vi "new-cacode.vi"() -> ()   [LabVIEW 2023]
uses:
  <vilib>/Utility/file.llb/Read Delimited Spreadsheet (string).vi
panel:
  out "all rows":string[][](array[string])
  in  "stop":bool
  in  "Run PRN Generator":bool
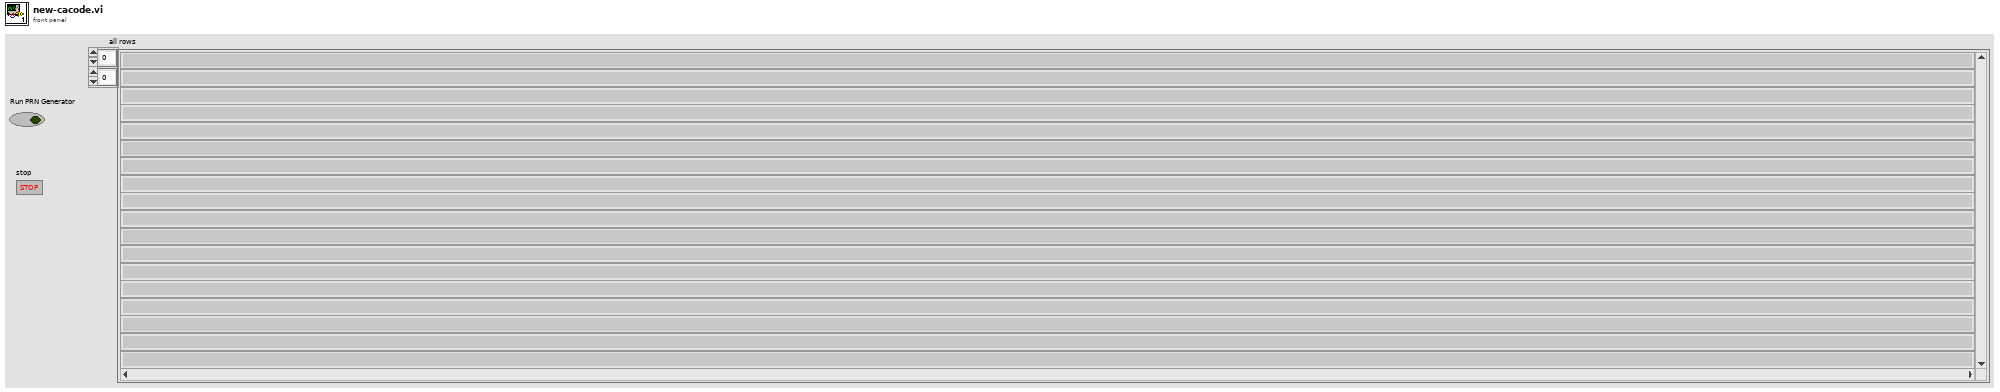
[diagram p1: front panel]
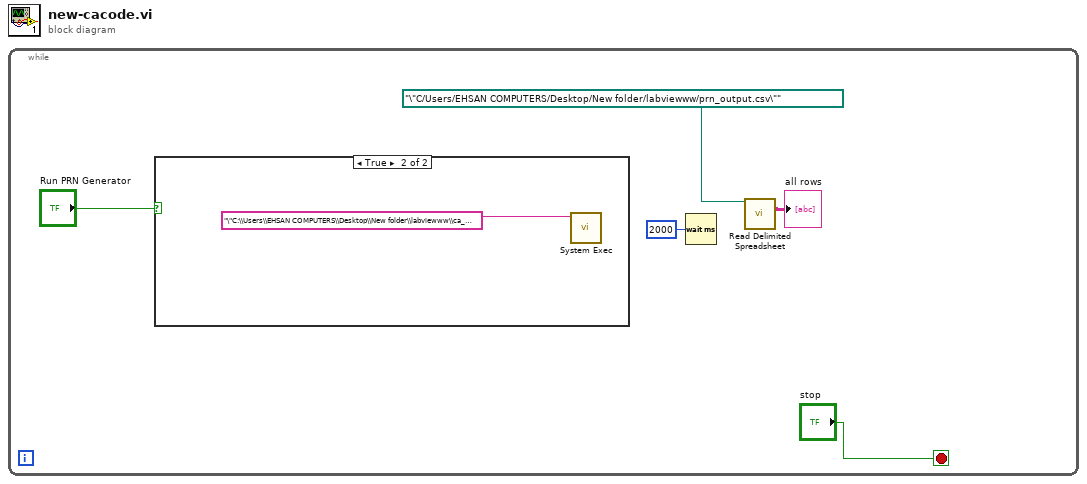
[diagram p0: block diagram]
diagram:
  n1 = while {
    stop <- "stop" stop-if-true
    n2 = case shown="True" "Run PRN Generator" {
      frame False {
      }
      frame True {
        n3 = call <vilib>:"System Exec.vi"("command line"="\"C:\\Users\\EHSAN COMPUTERS\\Desktop\\New folder\\labviewww\\ca_code.py\"") -> ()  [unwired: 7 in, 4 out]
      }
    }
    n4 = Wait (ms)(milliseconds to wait=u32 2000) -> ()  [unwired: 1 out]
    n5 = call-poly <vilib>:"Read Delimited Spreadsheet.vi"("file path (dialog if empty)"=path "/\"C/Users/EHSAN COMPUTERS/Desktop/New folder/labviewww/prn_output.csv\"") -> ("all rows"=→"all rows":string[][])  [unwired: 9 in, 5 out]
  }
